vi "Send Command.vi"(7 "VolatusAPI":refnum<class "VolatusAPI.lvclass">, 8 "error in (no error)":errorcluster, 10 "Value":dbl, 11 "DblPopupControl in":refnum<class "DblPopupControl.lvclass">) -> (0 "error out":errorcluster, 3 "DblPopupControl out":refnum<class "DblPopupControl.lvclass">)   [LabVIEW 2020, in "VolatusGUIElements.lvlib" / "DblPopupControl.lvclass"]
uses:
  DblPopupControl.lvclass
  Volatus/VolatusAPI/VolatusAPI.lvclass
  Cmd State.ctl
  DblPopupControl.lvclass/DblPopupControl.ctl
  messages/CmdAnalog/Class/Msg.lvclass/Msg.ctl
  Volatus/VolatusAPI/VolatusAPI.lvclass/VolatusAPI.ctl
  messages/CmdAnalog/Class/Msg.lvclass
  C:/dev/lv20CE/relink/lv-protoc/LV-Proto/Message/Message.lvclass
  lv-vecto/Vecto/TCPMessageService/Send Message.vi
  <vilib>/Utility/error.llb/Error Cluster From Error Code.vi
  lv-protoc/LV-Proto/Message/Message.lvclass
  Volatus/Numeric Command/Numeric Command.lvclass
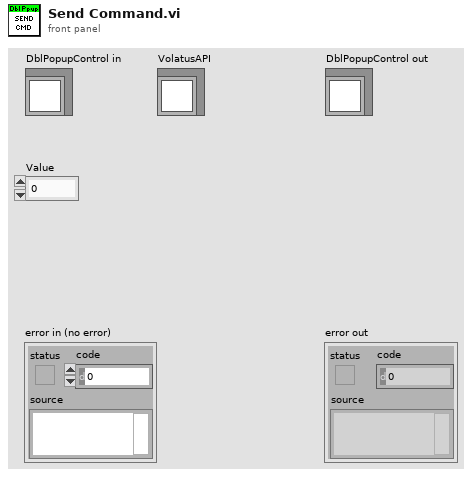
[diagram p1: front panel]
types:
  T1 = typedef "VolatusGUIElements.lvlib/DblPopupControl.lvclass/Cmd State.ctl" = cluster{"Commanding":bool, "Start":dbl, "Error":bool, "Value":dbl}
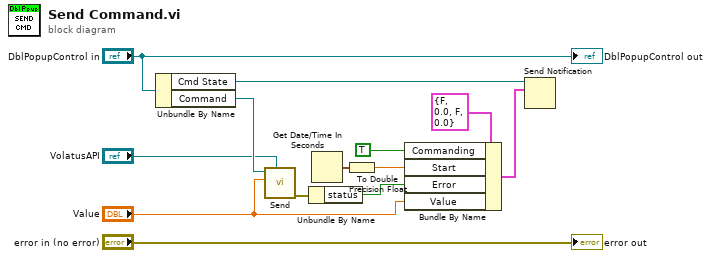
[diagram p0: block diagram]
diagram:
  n1 = Unbundle By Name("DblPopupControl in") -> ("Cmd State"=w11:refnum<notifier>, "Command"=w4:refnum<class "Numeric Command.lvclass">)
  n2 = call "Send.vi"("VolatusAPI"="VolatusAPI", "Value"="Value", "Numeric Command in"=w4) -> ("error out"=w1:errorcluster)  [unwired: 8 in]
  n3 = Unbundle By Name(w1) -> ("status"=w5:bool)
  n4 = Get Date/Time In Seconds() -> (seconds since 1Jan1904=w8:timestamp)
  n5 = To Double Precision Float(number=w8) -> (double precision float=w7:dbl)
  n6 = Bundle By Name(cluster=T1 {"Commanding"=FALSE, "Start"=0.0, "Error"=FALSE, "Value"=0.0} ("notification"), "Commanding"=TRUE, "Start"=w7, "Error"=w5, "Value"="Value") -> (w9:T1)
  n7 = Send Notification(notification=w9, notifier=w11) -> ()  [unwired: 1 in, 2 out]
  "error out" <- "error in (no error)"
  "DblPopupControl out" <- "DblPopupControl in"
